vi "Process Discovered Resources.vi"(9 "IO Resources in":T2[](array[typedef]), 10 "Software Resources in":T1[](array[typedef])) -> (1 "IO Resources out":T2[](array[typedef]), 2 "Software Resources out":T1[](array[typedef]))   [LabVIEW 2021, in "Acquisition.lvlib"]
doc: "Process the discovered resources and identify, correct, or drop entries as necessary."
uses:
  Acquisition.lvlib
  Host IO Resource.ctl
  Host Software Package.ctl
  381350fb-5328-4bce-9642-e04bcb1efc20.vi
  <vilib>/Array/Sort 2D Array - Pop Stack.vi
  <vilib>/Array/Sort 2D Array - Push Stack.vi
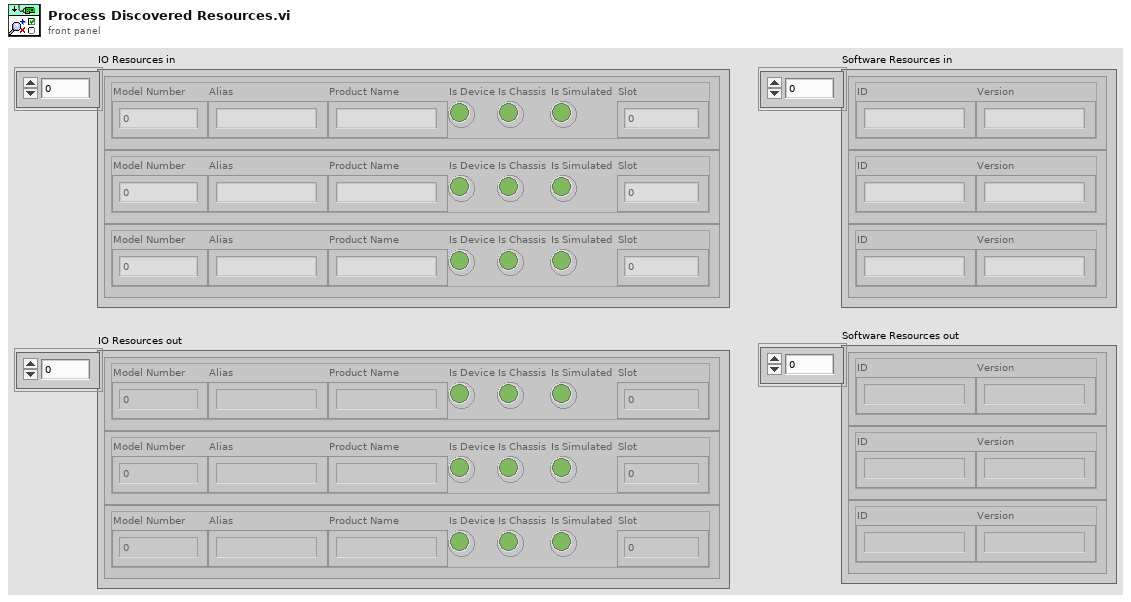
[diagram p1: front panel]
types:
  T1 = typedef "Acquisition.lvlib/Host Software Package.ctl" = cluster{"ID":string, "Version":string}
  T2 = typedef "Acquisition.lvlib/Host IO Resource.ctl" = cluster{"Model Number":u32, "Alias":string, "Product Name":string, "Is Device":bool, "Is Chassis":bool, "Is Simulated":bool, "Slot":i32}
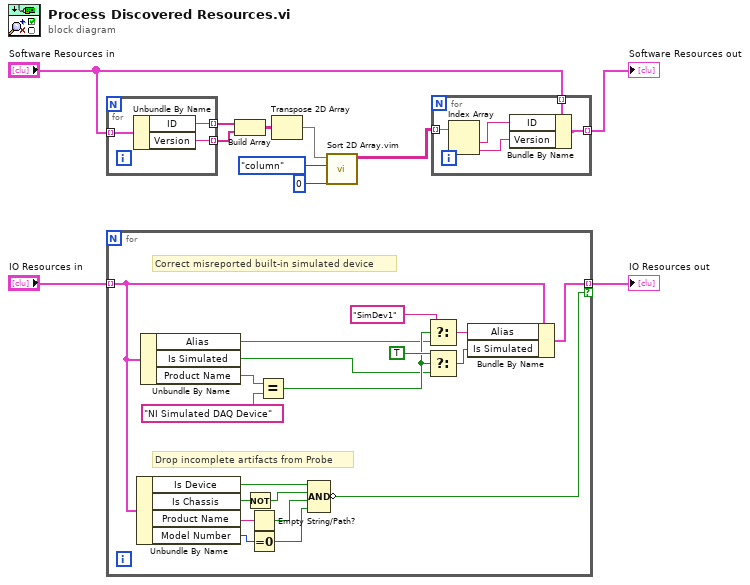
[diagram p0: block diagram]
diagram:
  n1 = for {
    tunnel: "Software Resources in" -> [w14] mode=indexing
    tunnel: [w13] -> w9 mode=indexing
    tunnel: [w12] -> w8 mode=indexing
    n2 = Unbundle By Name(w14) -> ("ID"=w13:string, "Version"=w12:string)
  }
  n3 = for {
    tunnel: "IO Resources in" -> [w29] mode=indexing
    tunnel: [w33] -> w10 mode=indexing if=w21
    # "Correct misreported built-in simulated device"
    # "Drop incomplete artifacts from Probe"
    n4 = Unbundle By Name(w29) -> ("Is Device"=w25:bool, "Is Chassis"=w26:bool, "Product Name"=w28:string, "Model Number"=w27:u32)
    n5 = Unbundle By Name(w29) -> ("Alias"=w17:string, "Is Simulated"=w15:bool, "Product Name"=w16:string)
    n6 = Not(x=w26) -> (.not. x?=w22:bool)
    n7 = Empty String/Path?(string/path=w28) -> (empty?=w23:bool)
    n8 = Equal To 0?(x=w27) -> (x = 0?=w24:bool)
    n9 = Equal?(x=w16, y="NI Simulated DAQ Device") -> (x = y?=w18:bool)
    n10 = Compound Arithmetic op=AND(w25, w22, w23, w24) -> (invert w21:bool)
    n11 = Select(t="SimDev1", s=w18, f=w17) -> (s? t:f=w20:string)
    n12 = Select(t=TRUE, s=w18, f=w15) -> (s? t:f=w32:bool)
    n13 = Bundle By Name(cluster=w29, "Alias"=w20, "Is Simulated"=w32) -> (w33:T2)
  }
  "IO Resources out" <- w10
  n14 = Build Array(w9, w8) -> (w7:string[][])
  n15 = Transpose 2D Array(2D array=w7) -> (transposed array=w1:string[][])
  n16 = call "Sort 2D Array.vim"("index"=0, "dimension to index (column)"=enum16{"column", "row"}."column", "2D array"=w1) -> ("sorted 2D array"=w4:string[][])  [unwired: 7 in, 1 out]
  n17 = for {
    tunnel: "Software Resources in" -> [w38] mode=indexing
    tunnel: w4 -> [w37] mode=indexing
    tunnel: [w34] -> w2 mode=indexing
    n18 = Index Array(array=w37) -> (element #1=w36:string, element #2=w35:string)  [unwired: 2 in]
    n19 = Bundle By Name(cluster=w38, "ID"=w36, "Version"=w35) -> (w34:T1)
  }
  "Software Resources out" <- w2
